vi "Update Byte Location.vi"(8 "error in (no error)":errorcluster, 9 "Size":T2, 11 "Channel in":refnum<class "Channel.lvclass">) -> (0 "error out":errorcluster, 1 "Location":T1, 3 "Channel out":refnum<class "Channel.lvclass">)   [LabVIEW 2026, in "Modbus.lvlib" / "Modbus.lvclass"]
uses:
  Modbus.lvclass
  <vilib>/FlexLogger/SDK/PluginSDK.lvlibp/PEFClasses/SDK/Channel/Channel.lvclass
  Types/Numeric Size.ctl
  Types/Numeric Location.ctl
  c3364b71-3b7c-4945-a381-b953504bea10.vi
  c3364b71-3b7c-4945-a381-b953504bea10.vi/407e0540-03f6-4363-afc5-a4b1f046ef19.vi
  c3364b71-3b7c-4945-a381-b953504bea10.vi/520d475a-7b95-4b20-931b-ccc2be82a762.vi
  Globals/Modbus Strings.vi
  <vilib>/FlexLogger/SDK/PluginSDK.lvlibp/PEFClasses/SDK/Channel/ParameterAccess/Read Enum.vi
  <vilib>/FlexLogger/SDK/PluginSDK.lvlibp/PEFClasses/SDK/Channel/ParameterAccess/Write Enum.vi
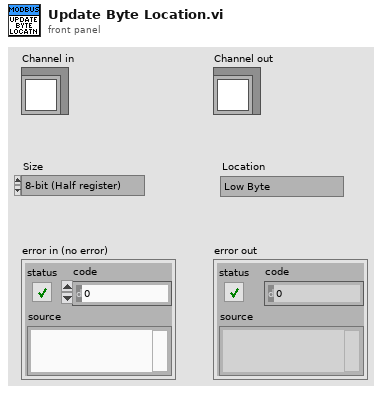
[diagram p1: front panel]
types:
  T1 = typedef "Modbus.lvlib/Modbus.lvclass/Numeric Location.ctl" = enum16{"Low Byte", "High Byte"}
  T2 = typedef "Modbus.lvlib/Modbus.lvclass/Numeric Size.ctl" = enum16{"8-bit (Half register)", "16-bit (One register)", "32-bit (Two registers)", "64-bit (Four registers)"}
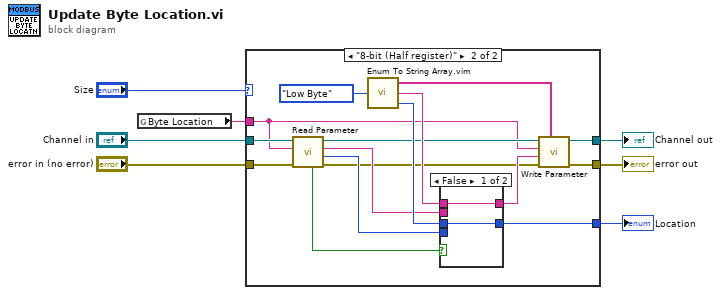
[diagram p0: block diagram]
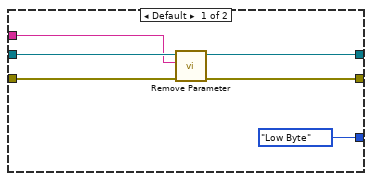
[diagram p2: hidden frame]
diagram:
  n1 = global read "Modbus Strings.vi" "Byte Location"() -> (w1:string)
  n2 = case shown="\"8-bit (Half register)\"" "Size" {
    tunnel: [Numeric_Location."Low Byte" ("Location") w26] -> w2
    tunnel: "error in (no error)" -> [w11 w18]
    tunnel: w1 -> [w8 w14]
    tunnel: "Channel in" -> [w12 w16]
    tunnel: [w9 w23] -> w7
    tunnel: [w10 w22] -> w6
    frame Default {
      n3 = call <vilib>:"Remove Parameter.vi"("error in (no error)"=w11, "Name"=w8, "Channel in"=w12) -> ("error out"=w9:errorcluster, "Channel out"=w10:refnum<class "Channel.lvclass">)  [unwired: 7 in]
    }
    frame "8-bit (Half register)" {
      n4 = call-poly <vilib>:"Read Parameter.vi"("error in (no error)"=w18, "Name"=w14, "Channel in"=w16) -> ("error out"=w17:errorcluster, "Index"=w19:i32, "Value"=w20:string, "Channel out"=w15:refnum<class "Channel.lvclass">, "Found"=w21:bool)  [unwired: 4 in]
      n5 = call "Enum To String Array.vim"("Enum in"=Numeric_Location."Low Byte" ("Location")) -> ("Selected Value out"=w27:T1, "Selected String out"=w28:string, "Strings out"=w25:string[])  [unwired: 2 in]
      n6 = case shown="False" w21 {
        tunnel: w28 -> [w31 _]
        tunnel: w27 -> [w30 _]
        tunnel: [w31 w33] -> w24
        tunnel: [w30 w32] -> w26
        tunnel: w19 -> [_ w32]
        tunnel: w20 -> [_ w33]
        frame False {
        }
        frame True {
        }
      }
      n7 = call-poly <vilib>:"Write Parameter.vi"("Possible Values"=w25, "error in (no error)"=w17, "Current Value"=w24, "Name"=w14, "Channel in"=w15) -> ("error out"=w23:errorcluster, "Channel out"=w22:refnum<class "Channel.lvclass">)  [unwired: 5 in]
    }
  }
  "error out" <- w7
  "Channel out" <- w6
  "Location" <- w2
